vi "PicoScopeospaAWG.vi"(0 "Handle In":i16=16384, 1 "General AWG Settings":T4={"Peak-to-Peak Voltage"=2.0, "Offset Voltage"=0.0, "Wave Type"=17, "Sweep Type"=0, "Cycles"=10, "Trigger Type"=0, "Trigger Source"=4, "sigGenEnabled"=TRUE, "Trigger Enabled"=FALSE, "autoTriggerPicoSeconds"=0} {"Trigger Source" items=["None"=0, "Scope Trigger"=1, "Software Trigger"=4, "Trigger Raw"=5]; "Trigger Type" items=["Rising", "Falling", "Gate High", "Gate Low"]; "Sweep Type" items=["Up", "Down", "Up-Down", "Down-Up"]; "Wave Type" items=["Sine"=17, "Square"=18, "Triangle"=19, "Ramp Up"=20, "Ramp Down"=21, "Sinc"=22, "Gaussian"=23, "Half Sine"=24, "DC"=1024, "PWM"=4096, "White Noise"=8193, "PRBS"=8194, "Arbitrary"=268435456]; "Offset Voltage" format="%#_6p"; "Peak-to-Peak Voltage" format="%#_6p"}, 2 "Standard Waveform Settings":T3={"(Start) Frequency"=1000.0, "Stop Frequency"=5000.0, "Increment"=1.0, "Dwell Time (seconds)"=0.001, "Sweep Enabled"=FALSE} {"Dwell Time (seconds)" format="%#_6p"; "Stop Frequency" min=0.03 max=1000000.0 format="%#_6p"; "(Start) Frequency" min=0.03 max=1000000.0 format="%#_6p"}, 3 "Arbitrary Waveform Settings":T2 {"Index Mode" items=["Single", "Dual", "Quad"]}, 11 "error in":errorcluster, 12 "Duty Cycle":T1={"Use Duty Cycle"=FALSE, "dutyCyclePercent"=20.0}) -> (4 "Handle Out":i16=16384, 13 "Trigger Source Out":u32=4, 14 "Arbitrary\nWaveform Graph":i16[](graph), 15 "error out":errorcluster)   [LabVIEW 2010]
doc: "This VI can be used to control the arbitrary waveform generator. Standard waveforms can be selected or arbitrary waveform can be selected under 'Wave Type'. There are three settings clusters: general settings that apply to both arbitrary and standard waveforms, settings that apply only to standard waveforms and settings that apply only to arbitrary waveforms. It is not necessary to connect all of these clusters if only using arbitrary waveforms or only using standard waveforms are required.\n\nWhen selecting arbitrary waveform, it is necessary to specify a text file containing the wave form. This text file should have a single value on each line in the range -1 to 1. For further information on the settings, see descriptions of ps3000aSetSigGenBuiltIn and ps3000aSetSigGenArbitrary."
uses:
  psospa.dll
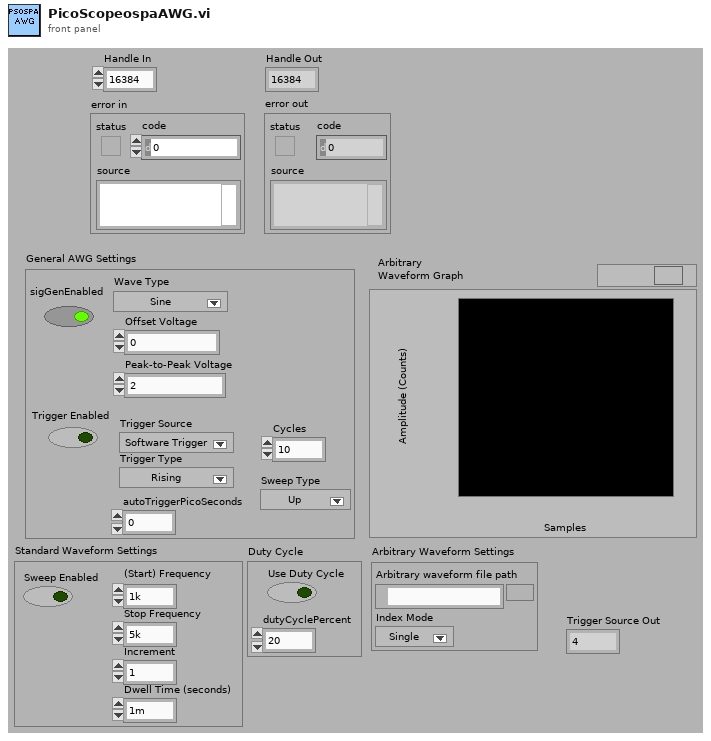
[diagram p1: front panel]
types:
  T1 = cluster{"Use Duty Cycle":bool, "dutyCyclePercent":dbl}
  T2 = cluster{"Arbirary waveform file path":path, "Index Mode":u32}
  T3 = cluster{"(Start) Frequency":dbl, "Stop Frequency":dbl, "Increment":dbl, "Dwell Time (seconds)":dbl, "Sweep Enabled":bool}
  T4 = cluster{"Peak-to-Peak Voltage":dbl, "Offset Voltage":dbl, "Wave Type":u32, "Sweep Type":u32, "Cycles":u64, "Trigger Type":u32, "Trigger Source":u32, "sigGenEnabled":bool, "Trigger Enabled":bool, "autoTriggerPicoSeconds":u64}
  T5 = cluster{"status":bool, "code":u32, "source":string}
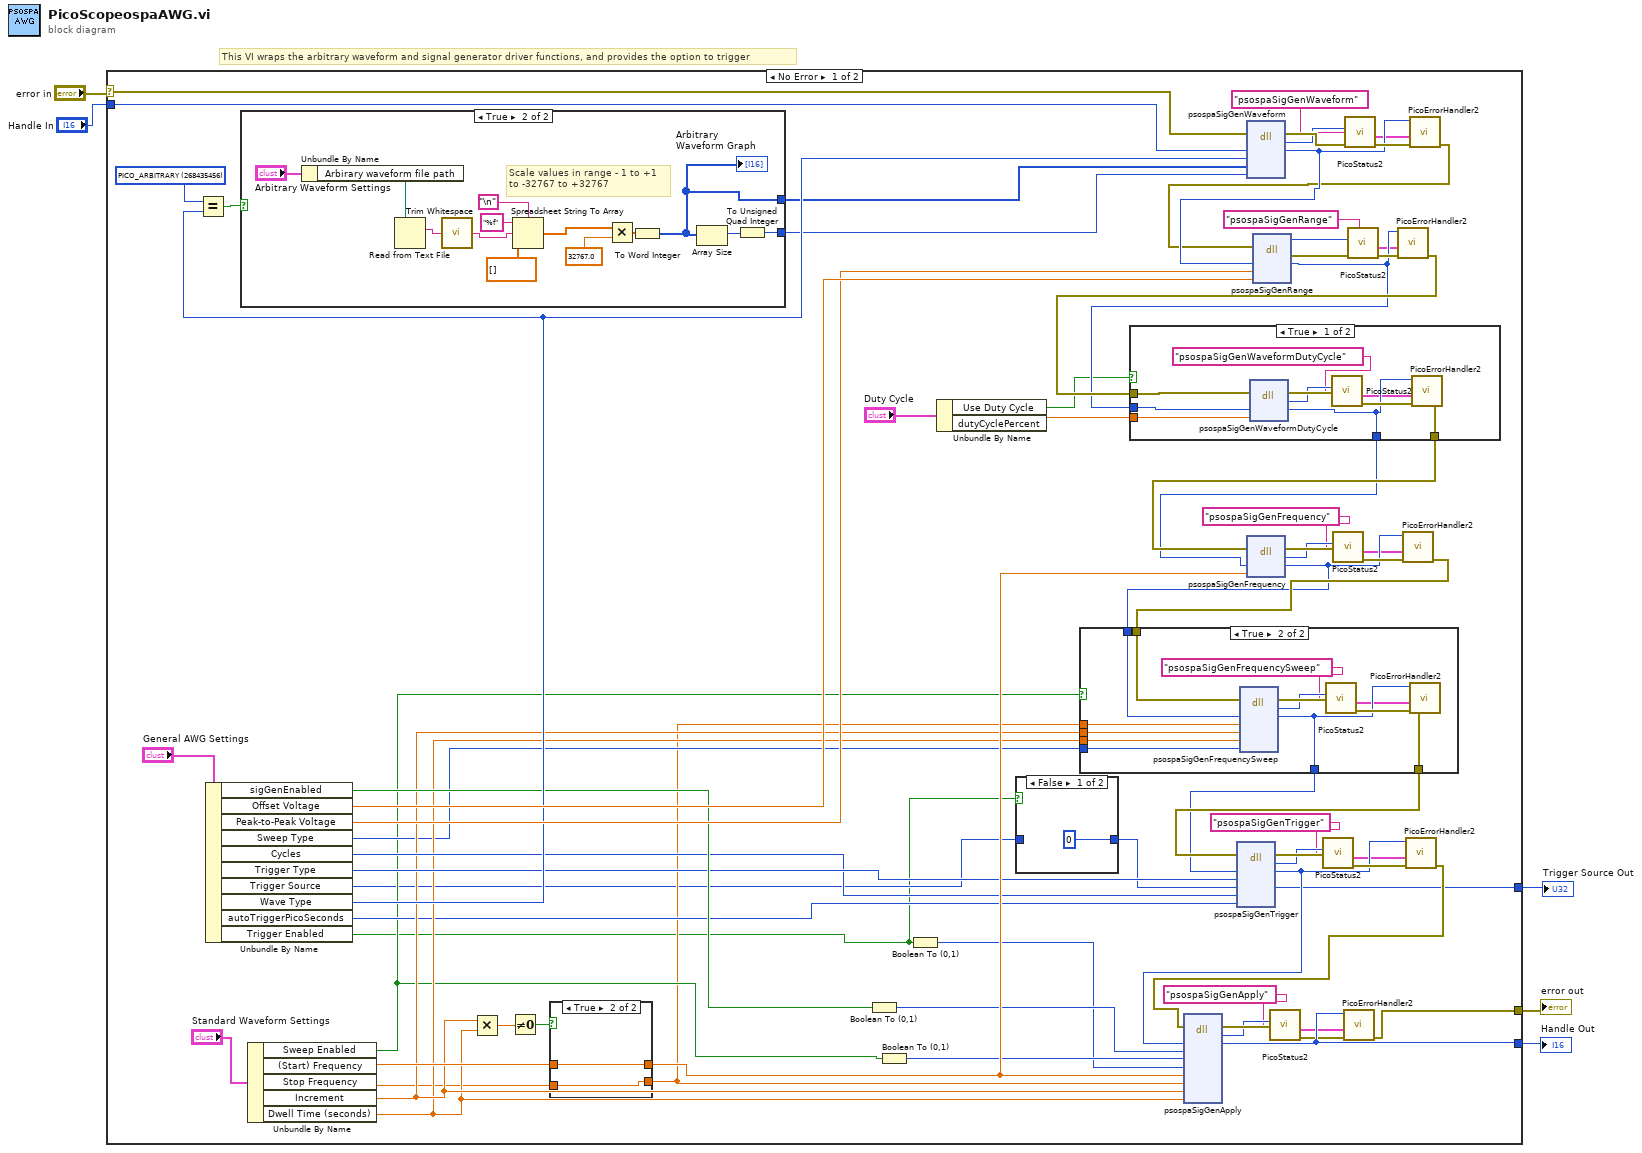
[diagram p0: block diagram]
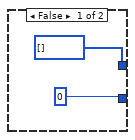
[diagram p4: hidden frame]
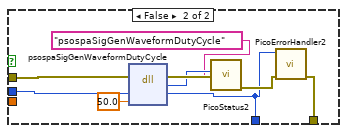
[diagram p5: hidden frame]
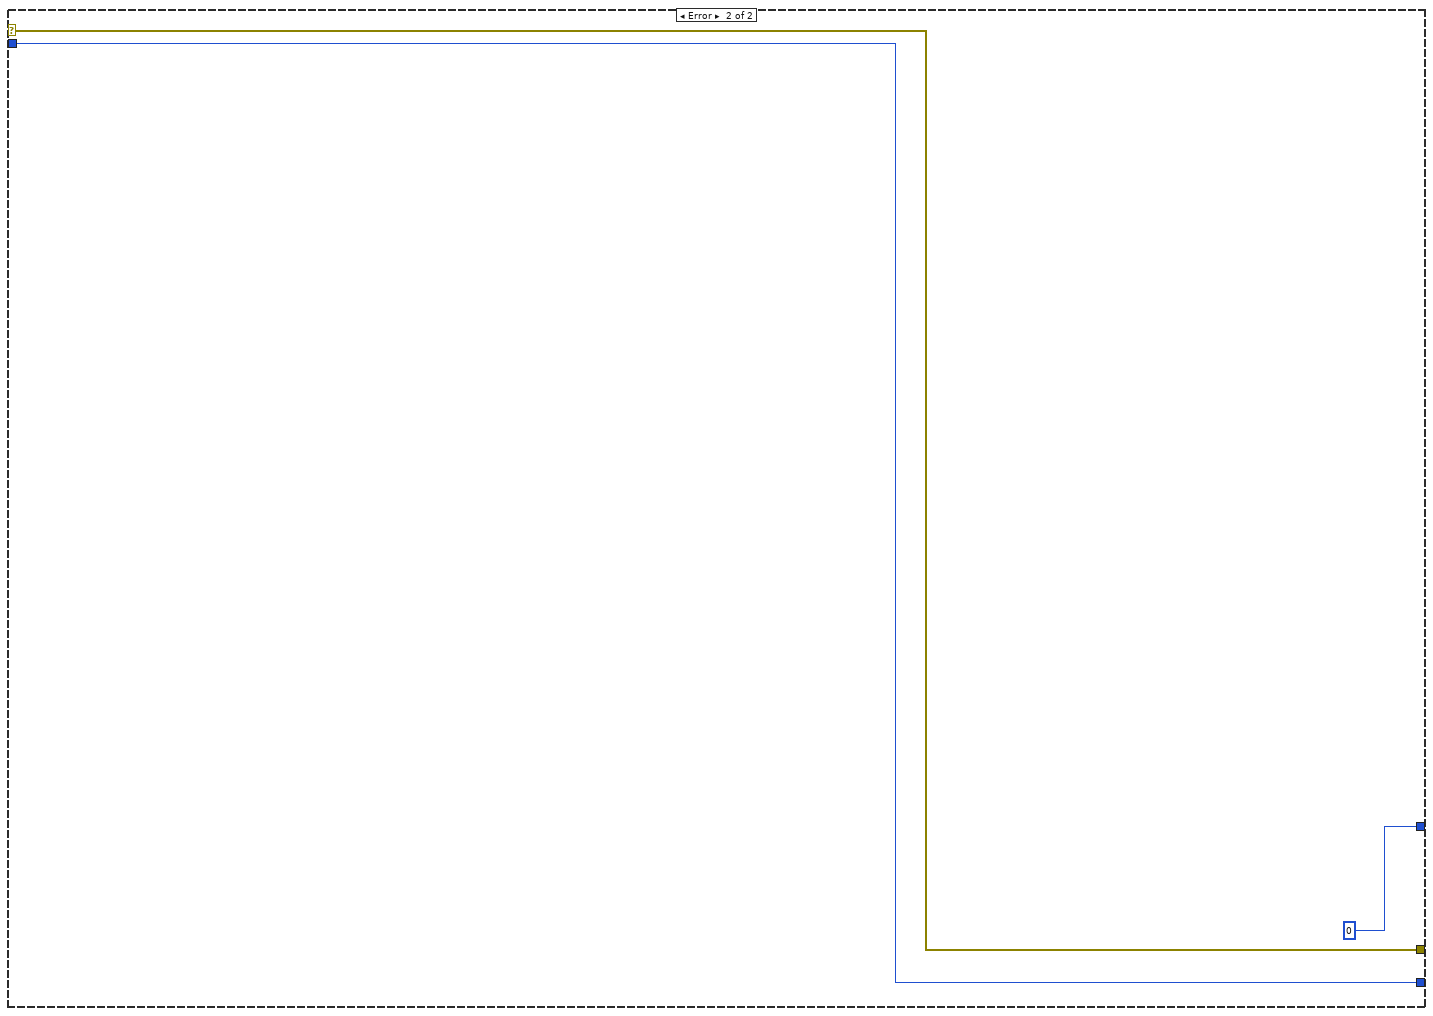
[diagram p7: hidden frame]
diagram:
  # "This VI wraps the arbitrary waveform and signal generator driver functions, and provides the option to trigger"
  n1 = case shown="No Error" "error in" {
    selector: "error in" -> [w74 w136]
    tunnel: [w68 w135] -> w5
    tunnel: "Handle In" -> [w79 w135]
    tunnel: [w67 w136] -> w3
    tunnel: [w14 0] -> w1
    frame No Error {
      w66 = u32 268435456 items=["PICO_ARBITRARY"=268435456]
      n2 = Unbundle By Name("General AWG Settings") -> ("sigGenEnabled"=w37:bool, "Offset Voltage"=w77:dbl, "Peak-to-Peak Voltage"=w76:dbl, "Sweep Type"=w18:u32, "Cycles"=w26:u64, "Trigger Type"=w27:u32, "Trigger Source"=w12:u32, "Wave Type"=w75:u32, "autoTriggerPicoSeconds"=w17:u64, "Trigger Enabled"=w11:bool)
      n3 = Equal?(x=w66, y=w75) -> (x = y?=w38:bool)
      n4 = case shown="True" w38 {
        tunnel: [i16[] [] ("buffer") w100] -> w47
        tunnel: [u64 0 ("bufferLenght") w99] -> w39
        frame False {
        }
        frame True {
          # "Scale values in range - 1 to +1 \nto -32767 to +32767"
          n5 = Unbundle By Name("Arbitrary Waveform Settings") -> ("Arbirary waveform file path"=w105:path)
          n6 = Read from Text File(file (use dialog)=w105) -> (text=w103:string)  [unwired: 3 in, 3 out]
          n7 = call <vilib>:"Trim Whitespace.vi"("string"=w103) -> ("trimmed string"=w102:string)  [unwired: 1 in]
          n8 = Spreadsheet String To Array(delimiter (Tab)="\n", format string="%f", spreadsheet string=w102, array type (2D Dbl)=dbl[] []) -> (array=w107:dbl[])
          n9 = Multiply(x=w107, y=32767.0 ("deltaPhaseIncrement")) -> (x*y=w104:dbl[])
          n10 = To Word Integer(number=w104) -> (16bit integer=w100:i16[])
          "Arbitrary\nWaveform Graph" <- w100
          n11 = Array Size(array=w100) -> (size(s)=w101:i32)
          n12 = To Unsigned Quad Integer(1:w101) -> (0:w99:u64)
        }
      }
      n13 = Unbundle By Name("Standard Waveform Settings") -> ("Sweep Enabled"=w16:bool, "(Start) Frequency"=w72:dbl, "Stop Frequency"=w23:dbl, "Increment"=w25:dbl, "Dwell Time (seconds)"=w24:dbl)
      n14 = Multiply(x=w25, y=w24) -> (x*y=w71:dbl)
      n15 = Not Equal To 0?(x=w71) -> (x != 0?=w70:bool)
      n16 = case shown="True" w70 {
        tunnel: [w131 w133] -> w15
        tunnel: w23 -> [_ w133]
        tunnel: w72 -> [w131 w132]
        tunnel: [w131 w132] -> w69
        frame False {
        }
        frame True {
        }
      }
      n17 = Boolean To (0,1)(Boolean=w37) -> (0, 1=w42:i16)
      n18 = Boolean To (0,1)(Boolean=w16) -> (0, 1=w41:i16)
      n19 = Boolean To (0,1)(Boolean=w11) -> (0, 1=w40:i16)
      n20 = Unbundle By Name("Duty Cycle") -> ("Use Duty Cycle"=w35:bool, "dutyCyclePercent"=w34:dbl)
      n21 = case shown="False" w11 {
        tunnel: [u32 0 ("Trigger Source") w81] -> w13
        tunnel: w12 -> [_ w81]
        frame False {
        }
        frame True {
        }
      }
      n22 = dll-call lib="psospa.dll" fn="psospaSigGenWaveform" ("ps3000.dll:_ps3000_open_unit@0")(error in=w74, "handle"=w79, "waveType"=w75, "buffer"=w47, "bufferLenght"=w39) -> (error out=w63:errorcluster, "PICO_STATUS"=w55:u32, "handle"=w60:i16)  [unwired: 5 in, 1 out]
      n23 = call "PicoStatus2.vi"("PICO source"="psospaSigGenWaveform" ("source"), "Error in"=w63, "PICO STATUS"=w55) -> ("error out"=w62:errorcluster, "PICO_STATUS out"=w10:T5)  [unwired: 5 in]
      n24 = call "PicoErrorHandler2.vi"("error in (no error)"=w62, "PICO_STATUS in"=w10, "handle In"=w60) -> ("error out"=w59:errorcluster)  [unwired: 8 in]
      n25 = dll-call lib="psospa.dll" fn="psospaSigGenRange" ("ps3000.dll:_ps3000_open_unit@0")(error in=w59, "handle"=w60, "peakToPeakVolts"=w76, "offsetVolts"=w77) -> (error out=w58:errorcluster, "PICO_STATUS"=w56:u32, "handle"=w53:i16)  [unwired: 4 in, 1 out]
      n26 = call "PicoStatus2.vi"("PICO source"="psospaSigGenRange" ("source"), "Error in"=w58, "PICO STATUS"=w56) -> ("error out"=w57:errorcluster, "PICO_STATUS out"=w9:T5)  [unwired: 5 in]
      n27 = call "PicoErrorHandler2.vi"("error in (no error)"=w57, "PICO_STATUS in"=w9, "handle In"=w53) -> ("error out"=w54:errorcluster)  [unwired: 8 in]
      n28 = case shown="True" w35 {
        tunnel: w54 -> [w118 w127]
        tunnel: w53 -> [w117 w126]
        tunnel: [w116 w125] -> w51
        tunnel: [w115 w124] -> w50
        tunnel: w34 -> [w113 _]
        frame True {
          n29 = dll-call lib="psospa.dll" fn="psospaSigGenWaveformDutyCycle" ("ps3000.dll:_ps3000_open_unit@0")(error in=w118, "handle"=w117, "dutyCyclePercent"=w113) -> (error out=w121:errorcluster, "PICO_STATUS"=w120:u32, "handle"=w115:i16)  [unwired: 3 in, 1 out]
          n30 = call "PicoStatus2.vi"("PICO source"="psospaSigGenWaveformDutyCycle" ("source"), "Error in"=w121, "PICO STATUS"=w120) -> ("error out"=w119:errorcluster, "PICO_STATUS out"=w112:T5)  [unwired: 5 in]
          n31 = call "PicoErrorHandler2.vi"("error in (no error)"=w119, "PICO_STATUS in"=w112, "handle In"=w115) -> ("error out"=w116:errorcluster)  [unwired: 8 in]
        }
        frame False {
          n32 = dll-call lib="psospa.dll" fn="psospaSigGenWaveformDutyCycle" ("ps3000.dll:_ps3000_open_unit@0")(error in=w127, "handle"=w126, "dutyCyclePercent"=50.0) -> (error out=w130:errorcluster, "PICO_STATUS"=w129:u32, "handle"=w124:i16)  [unwired: 3 in, 1 out]
          n33 = call "PicoStatus2.vi"("PICO source"="psospaSigGenWaveformDutyCycle" ("source"), "Error in"=w130, "PICO STATUS"=w129) -> ("error out"=w128:errorcluster)  [unwired: 5 in, 1 out]
          n34 = call "PicoErrorHandler2.vi"("error in (no error)"=w128, "handle In"=w124) -> ("error out"=w125:errorcluster)  [unwired: 9 in]
        }
      }
      n35 = dll-call lib="psospa.dll" fn="psospaSigGenFrequency" ("ps3000.dll:_ps3000_open_unit@0")(error in=w51, "handle"=w50, "frequencyHz"=w69) -> (error out=w65:errorcluster, "PICO_STATUS"=w64:u32, "handle"=w21:i16)  [unwired: 3 in, 1 out]
      n36 = call "PicoStatus2.vi"("PICO source"="psospaSigGenFrequency" ("source"), "Error in"=w65, "PICO STATUS"=w64) -> ("error out"=w52:errorcluster, "PICO_STATUS out"=w8:T5)  [unwired: 5 in]
      n37 = call "PicoErrorHandler2.vi"("error in (no error)"=w52, "PICO_STATUS in"=w8, "handle In"=w21) -> ("error out"=w22:errorcluster)  [unwired: 8 in]
      n38 = case shown="True" w16 {
        tunnel: w25 -> [_ w92]
        tunnel: w24 -> [_ w91]
        tunnel: w15 -> [_ w90]
        tunnel: w22 -> [w82 w89]
        tunnel: w21 -> [w83 w88]
        tunnel: [w82 w87] -> w20
        tunnel: [w83 w86] -> w19
        tunnel: w18 -> [_ w85]
        frame False {
        }
        frame True {
          n39 = dll-call lib="psospa.dll" fn="psospaSigGenFrequencySweep" ("ps3000.dll:_ps3000_open_unit@0")(error in=w89, "handle"=w88, "stopFrequencyHz"=w90, "frequencyIncrement"=w92, "dwellTimeSeconds"=w91, "sweepType"=w85) -> (error out=w96:errorcluster, "PICO_STATUS"=w95:u32, "handle"=w86:i16)  [unwired: 6 in, 1 out]
          n40 = call "PicoStatus2.vi"("PICO source"="psospaSigGenFrequencySweep" ("source"), "Error in"=w96, "PICO STATUS"=w95) -> ("error out"=w94:errorcluster, "PICO_STATUS out"=w84:T5)  [unwired: 5 in]
          n41 = call "PicoErrorHandler2.vi"("error in (no error)"=w94, "PICO_STATUS in"=w84, "handle In"=w86) -> ("error out"=w87:errorcluster)  [unwired: 8 in]
        }
      }
      n42 = dll-call lib="psospa.dll" fn="psospaSigGenTrigger" ("ps3000.dll:_ps3000_open_unit@0")(error in=w20, "handle"=w19, "triggerType"=w27, "triggerSource"=w13, "cycles"=w26, "autoTriggerPicoSeconds"=w17) -> (error out=w33:errorcluster, "PICO_STATUS"=w32:u32, "handle"=w28:i16, "triggerSource"=w14:u32)  [unwired: 5 in, 1 out]
      n43 = call "PicoStatus2.vi"("PICO source"="psospaSigGenTrigger" ("source"), "Error in"=w33, "PICO STATUS"=w32) -> ("error out"=w31:errorcluster, "PICO_STATUS out"=w7:T5)  [unwired: 5 in]
      n44 = call "PicoErrorHandler2.vi"("error in (no error)"=w31, "PICO_STATUS in"=w7, "handle In"=w28) -> ("error out"=w29:errorcluster)  [unwired: 8 in]
      n45 = dll-call lib="psospa.dll" fn="psospaSigGenApply" ("ps3000.dll:_ps3000_open_unit@0")(error in=w29, "handle"=w28, "sigGenEnabled"=w42, "sweepEnabled"=w41, "triggerEnabled"=w40, "frequency"=w69, "stopFrequency"=w15, "frequencyIncrement"=w25, "dwellTime"=w24) -> (error out=w46:errorcluster, "PICO_STATUS"=w45:u32, "handle"=w68:i16)  [unwired: 9 in, 1 out]
      n46 = call "PicoStatus2.vi"("PICO source"="psospaSigGenApply" ("source"), "Error in"=w46, "PICO STATUS"=w45) -> ("error out"=w44:errorcluster, "PICO_STATUS out"=w6:T5)  [unwired: 5 in]
      n47 = call "PicoErrorHandler2.vi"("error in (no error)"=w44, "PICO_STATUS in"=w6, "handle In"=w68) -> ("error out"=w67:errorcluster)  [unwired: 8 in]
    }
    frame Error {
    }
  }
  "Handle Out" <- w5
  "error out" <- w3
  "Trigger Source Out" <- w1
